vi "updateTable2.vi"(4 "颜色盒":u32(colorbox)=32768, 6 "类型":enum16{"无", "单格", "整行", "整列"}(ring)=enum."单格", 8 "error in (no error)":errorcluster caption="错误输入（无错误）", 9 "Value":string, 10 "Row":i32, 11 "Col":i32=5) -> (0 "error out":errorcluster caption="错误输出")   [LabVIEW 2025]
uses:
  global.vi
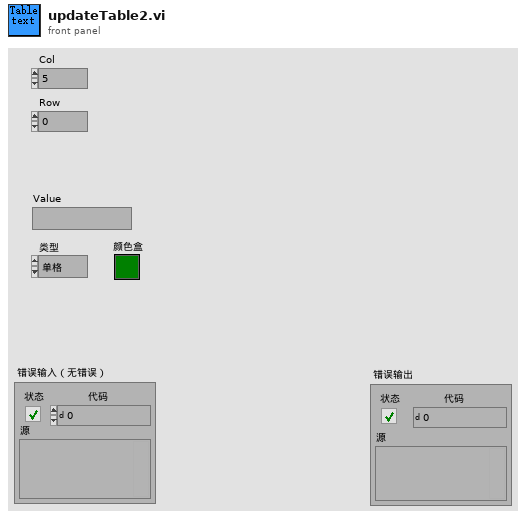
[diagram p1: front panel]
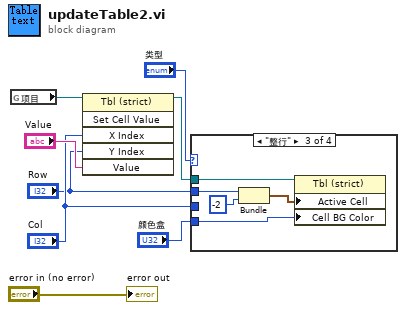
[diagram p0: block diagram]
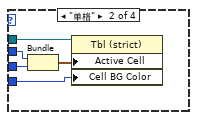
[diagram p3: hidden frame]
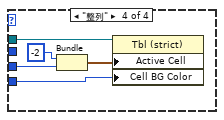
[diagram p4: hidden frame]
diagram:
  n1 = global read "global.vi" "项目"() -> (w7:refnum<vi>)
  n2 = invoke class="Tbl (strict)" method="Set Cell Value"(reference=w7, "X Index"="Col", "Y Index"="Row", "Value"="Value") -> (reference out=w5:refnum<vi>)  [unwired: 2 in, 5 out]
  n3 = case shown="\"整行\"" "类型" {
    tunnel: w5 -> [_ w12 w17 w22]
    tunnel: "Col" -> [_ w9 _ w19]
    tunnel: "Row" -> [_ w10 w15 _]
    tunnel: "颜色盒" -> [_ w11 w16 w21]
    frame "无", Default {
    }
    frame "单格" {
      n4 = Bundle("Row"=w10, "Col"=w9) -> (w13:cluster{"Row":i32, "Col":i32})  [unwired: 1 in]
      n5 = property class="Tbl (strict)"(reference=w12, "Active Cell"=w13, "Cell BG Color"=w11) -> ()  [unwired: 1 in, 2 out]
    }
    frame "整行" {
      n6 = Bundle("Row"=w15, -2) -> (w18:cluster{"Row":i32, i32})  [unwired: 1 in]
      n7 = property class="Tbl (strict)"(reference=w17, "Active Cell"=w18, "Cell BG Color"=w16) -> ()  [unwired: 1 in, 2 out]
    }
    frame "整列" {
      n8 = Bundle(-2, "Col"=w19) -> (w23:cluster{i32, "Col":i32})  [unwired: 1 in]
      n9 = property class="Tbl (strict)"(reference=w22, "Active Cell"=w23, "Cell BG Color"=w21) -> ()  [unwired: 1 in, 2 out]
    }
  }
  "error out" <- "error in (no error)"
